vi "VirtualATE_V2.vi"() -> ()   [LabVIEW 2026]
uses:
  <vilib>/NI/Modbus Library/API/Modbus API.lvclass/Modbus API.ctl
  <vilib>/NI/Modbus Library/Transmission Data Unit/Transmission Data Unit.lvclass/Transmission Data Unit.ctl
  <vilib>/NI/Modbus Library/Transmission Data Unit/Write Unit ID.vi
  <vilib>/NI/Modbus Library/API/Read Transmission Data Unit.vi
  <vilib>/NI/Modbus Library/API/Write Transmission Data Unit.vi
  <vilib>/NI/Modbus Library/API/Master/Modbus Master.lvclass
  C:/Program Files/National Instruments/LabVIEW 2026/vi.lib/NI/Modbus Library/API/Modbus API.lvclass
  <vilib>/NI/Modbus Library/API/Wrapper/Create TCP Master.vi
  <vilib>/NI/Modbus Library/API/Wrapper/API Main.lvlib
panel:
  out "PLC_HB_TIMEOUT":bool
  out "PLC_HB_AGE_MS":u32
  out "PLC_LIVE_OK":bool
  out "STATE_ELAPSED_MS":u32
  out "처리 메시지":string
  out "ATE_READY":bool
  out "ACTIVE_RESULT":u16
  out "ACTIVE_ID":u16
  out "ATE_STATE":u16
  out "PLC_LIVE_COUNTER":u16
  out "PLC_ACCEPTED_ID":u16
  out "PLC_RX_RESPONSE_ID":u16
  out "PLC_RX_DONE":u16
  out "PLC_RX_RESULT":u16
  in  "검사 결과 선택":enum16{"PASS", "FAIL", "RETEST"}(ring)
  out "바깥 Tick Count(ms)":u32
  in  "ATE 읽기 정지":bool
  out "ALARM_CODE":u16
  out "SEQ_STATE":u16
  out "TEEST_RESULT_LATCH":u16
  out "ATE_DONE":u16
  out "ATE_RESPONSE_ID":u16
  out "ATE_RESULT":u16
  out "ATE_REQUEST_ID":u16
  out "ATE_REQUEST":u16
  out "마지막 Modbus 읽기 정상":bool
  out "수신 레지스터":u16[](array[numeric])
  out "error out":errorcluster
  in  "Unit ID":u8
  in  "Port":u16
  in  "Server IP":string
  # "0 ATE_LINK_TEST\n1 ATE_REQUEST\n2 ATE_REQUEST_ID\n3 ATE_RESULT\n4 ATE_RESPONSE_ID\n5 ATE_DONE\n6 TEST_RESULT_LATCH\n7 SEQ_STATE\n8 ALARM_CODE"
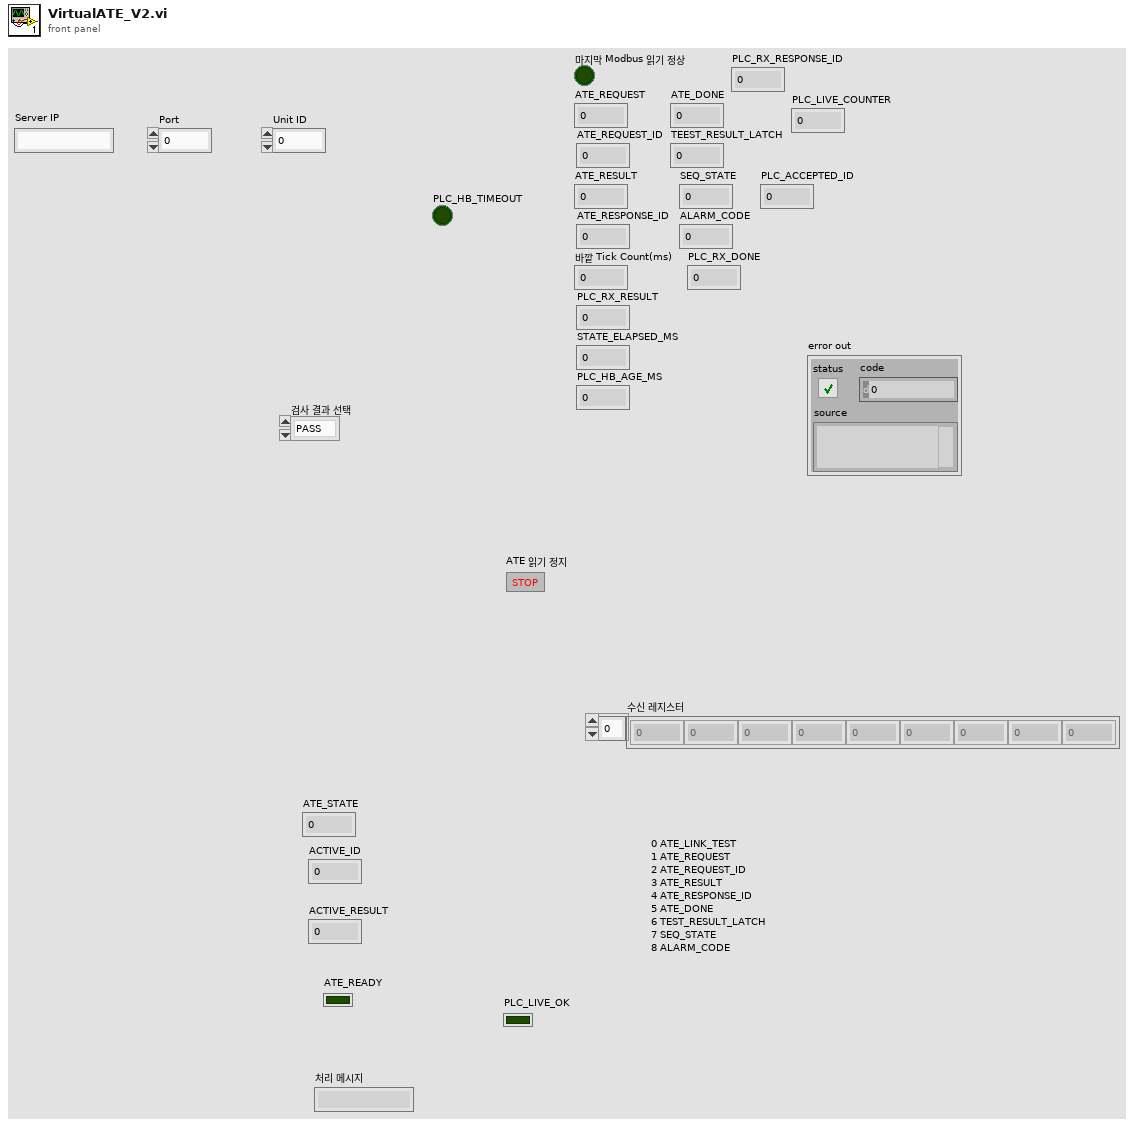
[diagram p1: front panel]
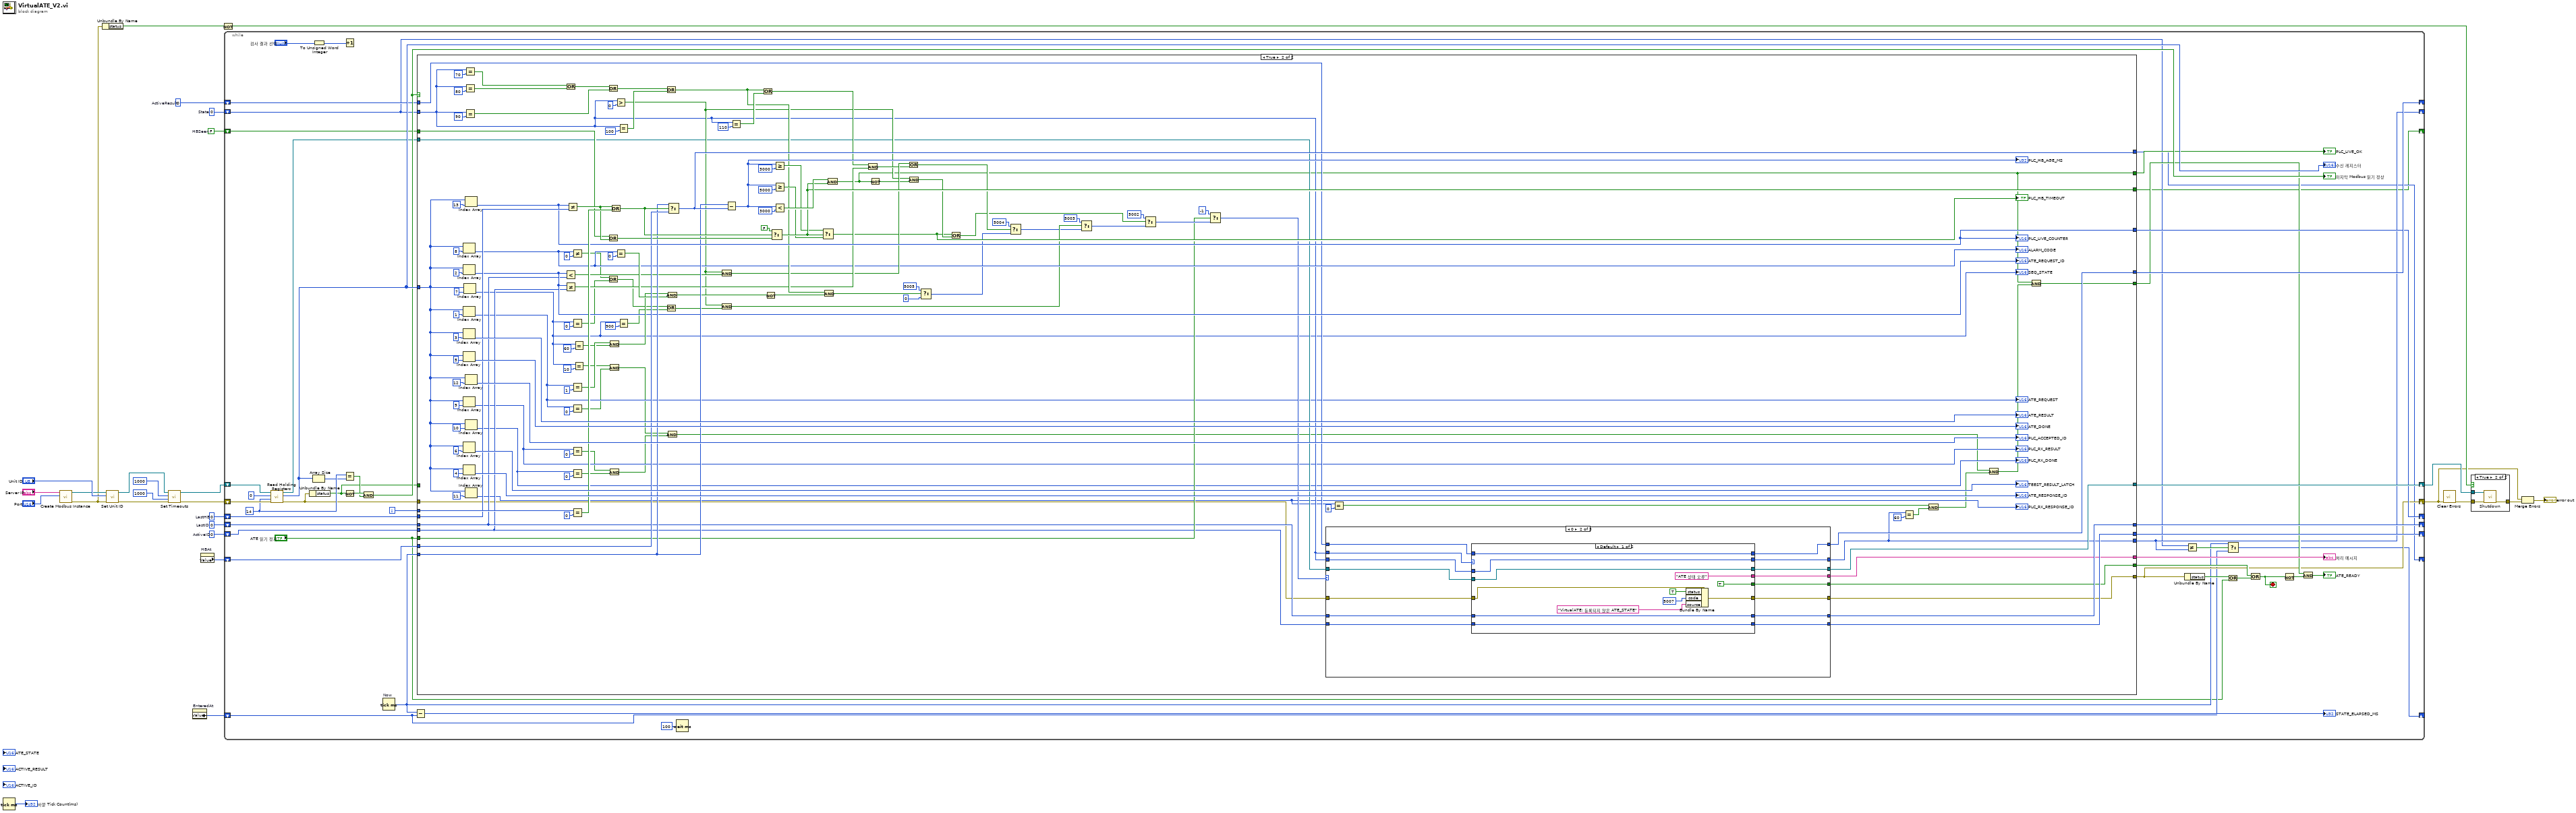
[diagram p0: block diagram]
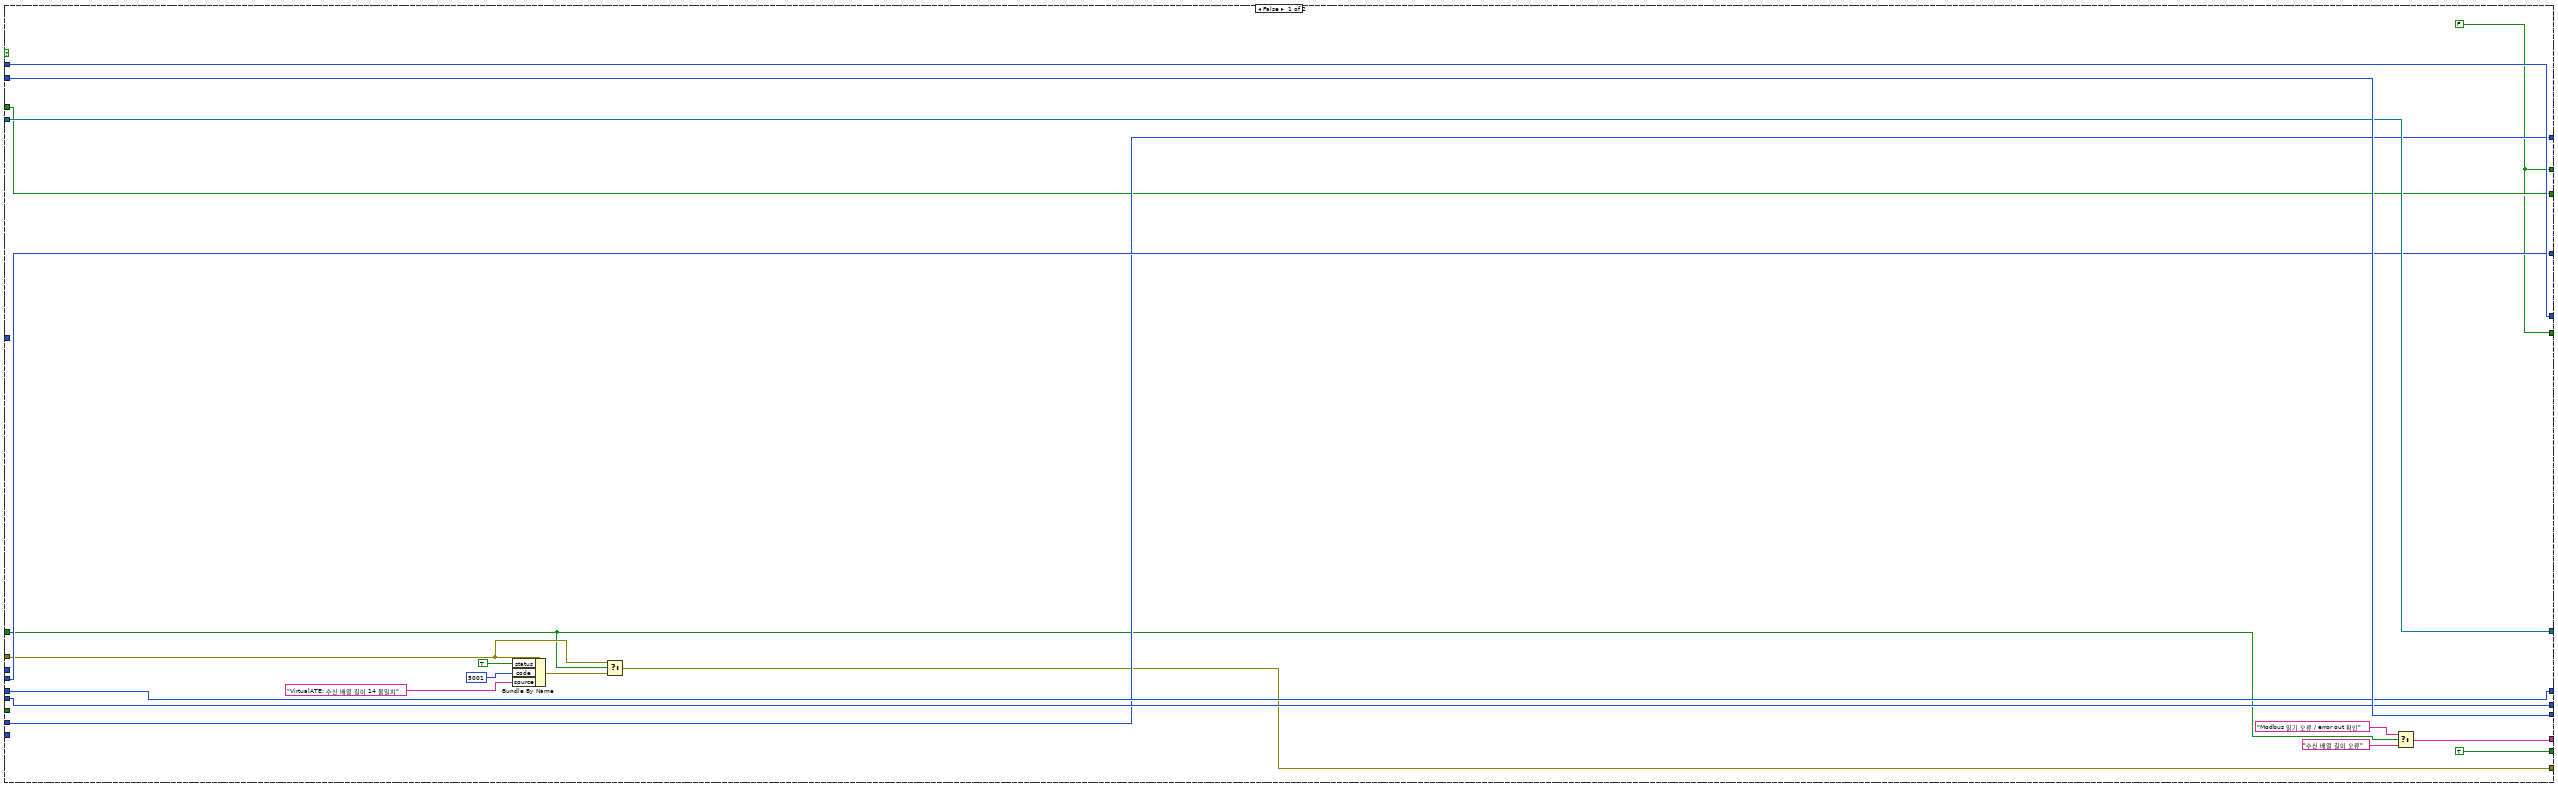
[diagram p3: hidden frame]
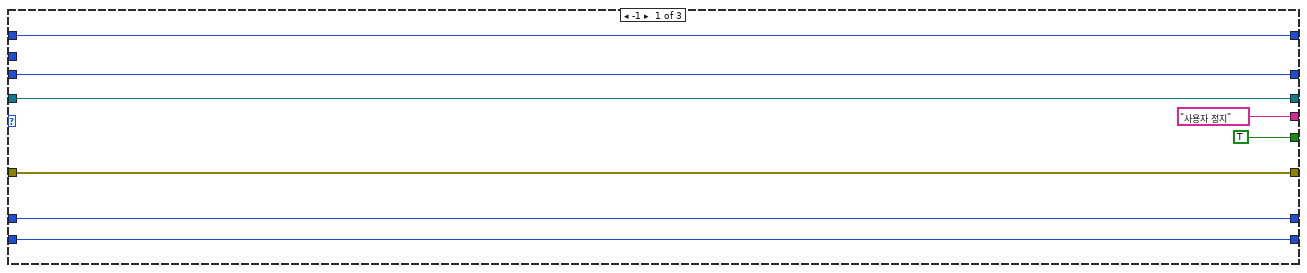
[diagram p4: hidden frame]
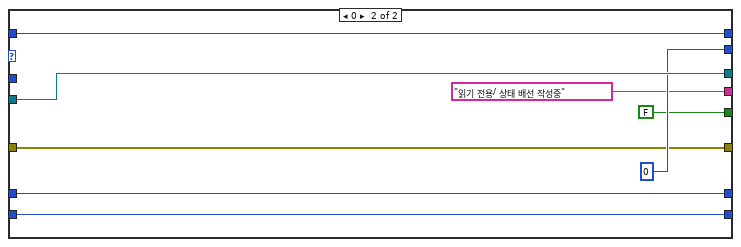
[diagram p5: hidden frame]
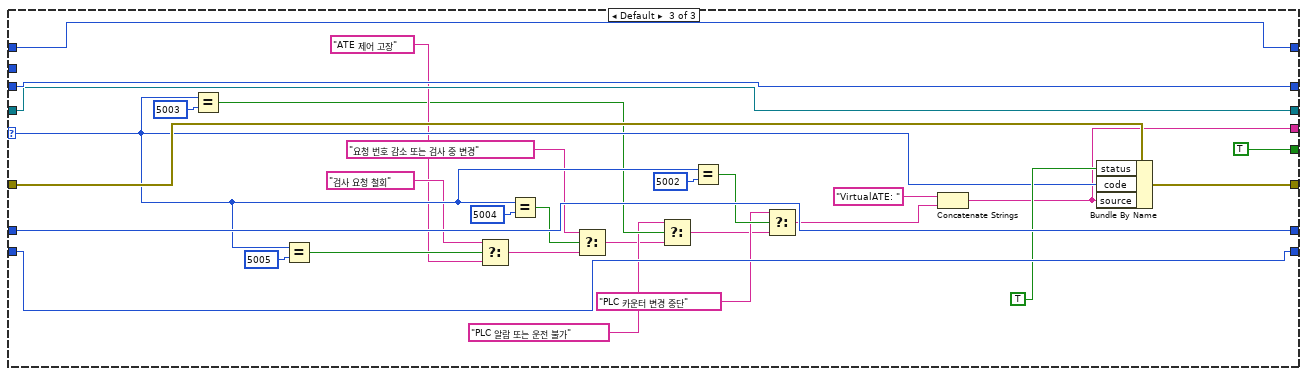
[diagram p6: hidden frame]
diagram:
  w9 = FALSE  # HBSeen
  w4 = u16 0  # LastHB
  w5 = u16 0  # ActiveResult
  w6 = u16 0  # ActiveID
  w7 = u16 0  # LastID
  w8 = u16 0  # State
  n1 = Tick Count (ms)() -> (millisecond timer value=→"바깥 Tick Count(ms)":u32)
  n2 = call-poly <vilib>:"Create Modbus Instance.vi"("port (502)"="Port", "address"="Server IP") -> ("error out"=w17:errorcluster, "TCP master instance"=w22:refnum<class "Modbus Master.lvclass">)  [unwired: 8 in]
  n3 = Unbundle By Name(w17) -> ("status"=w16:bool)
  n4 = call <vilib>:"Set Unit ID.vi"("error in"=w17, "unit ID"="Unit ID", "Modbus master in"=w22) -> ("error out"=w20:errorcluster, "Modbus master out"=w21:refnum<class "Modbus Master.lvclass">)  [unwired: 7 in]
  n5 = call <vilib>:"Set Timeouts.vi"("error in"=w20, "write operation timeout"=1000, "read operation timeout"=1000, "Modbus master in"=w21) -> ("error out"=w18:errorcluster, "Modbus master out"=w19:refnum<class "Modbus Master.lvclass">)  [unwired: 6 in]
  n6 = property on="EnteredAt" class="DigNum (strict)"() -> ("Value"=w2:u32)  [unwired: 2 in, 2 out]
  n7 = property on="HBAt" class="DigNum (strict)"() -> ("Value"=w1:u32)  [unwired: 2 in, 2 out]
  n8 = Not(x=w16) -> (.not. x?=w15:bool)
  n9 = while {
    shift-right: [w42] -> w11
    shift-left: w18 -> [w71]
    shift-right: [w54] -> w14
    shift-left: w19 -> [w72]
    shift-right: [w34] -> _
    shift-left: w8 -> [w33]
    shift-right: [w60] -> _
    shift-left: w7 -> [w61]
    shift-right: [w58] -> _
    shift-left: w6 -> [w59]
    shift-right: [w56] -> _
    shift-left: w5 -> [w57]
    shift-right: [w31] -> _
    shift-left: w1 -> [w50]
    shift-right: [w51] -> _
    shift-left: w4 -> [w52]
    shift-right: [w36] -> _
    shift-left: w2 -> [w32]
    shift-right: [w30] -> _
    shift-left: w9 -> [w49]
    i -> [w37]
    stop <- w39 stop-if-true
    w70 = u16 14 ("number of inputs")
    n10 = call-dynamic "Read Holding Registers.vi"("error in"=w71, "number of inputs"=w70, "starting address"=u16 0, "Modbus master in"=w72) -> ("error out"=w53:errorcluster, "register values"=w66:u16[], "Modbus master out"=w55:refnum<class "Modbus Master.lvclass">)  [unwired: 5 in]
    "수신 레지스터" <- w66
    n11 = Unbundle By Name(w53) -> ("status"=w48:bool)
    n12 = Array Size(array=w66) -> (size(s)=w69:i32)
    n13 = To Unsigned Word Integer(number="검사 결과 선택") -> (unsigned 16bit integer=w64:u16)
    n14 = Increment(x=w64) -> ()  [unwired: 1 out]
    n15 = Equal?(x=w70, y=w69) -> (x = y?=w67:bool)
    n16 = Not(x=w48) -> (.not. x?=w68:bool)
    n17 = And(x=w68, y=w67) -> (x .and. y?=w65:bool)
    "마지막 Modbus 읽기 정상" <- w65
    n18 = Tick Count (ms) "Now"() -> (millisecond timer value=w29:u32)
    n19 = Subtract(x=w29, y=w32) -> (x-y=→"STATE_ELAPSED_MS":u32)
    n20 = case shown="True" w65 {
      tunnel: w66 -> [_ w218]
      tunnel: w33 -> [w94 w120]
      tunnel: [w94 w109] -> w34
      tunnel: w61 -> [w93 w132]
      tunnel: [w93 w131] -> w60
      tunnel: w59 -> [w92 w130]
      tunnel: [w92 w129] -> w58
      tunnel: w57 -> [w91 w128]
      tunnel: [w91 w127] -> w56
      tunnel: w55 -> [w90 w126]
      tunnel: [w90 w125] -> w54
      tunnel: w53 -> [w82 w124]
      tunnel: [w76 w123] -> w42
      tunnel: w52 -> [w89 w209]
      tunnel: [w89 w205] -> w51
      tunnel: w50 -> [w88 w203]
      tunnel: [w88 w204] -> w31
      tunnel: w49 -> [w87 w206]
      tunnel: [w87 w193] -> w30
      tunnel: w48 -> [w80 _]
      tunnel: [TRUE w121] -> w46
      tunnel: [w77 w122] -> w45
      tunnel: [w75 w95] -> w43
      tunnel: [w75 w96] -> w38
      tunnel: w37 -> [_ w211]
      tunnel: w29 -> [_ w197]
      tunnel: "ATE 읽기 정지" -> [_ w134]
      frame False {
        w75 = FALSE
        n21 = Bundle By Name(cluster=w82, "status"=TRUE, "code"=5001, "source"="VirtualATE: 수신 배열 길이 14 불일치") -> (w83:errorcluster)
        n22 = Select(t=w82, s=w80, f=w83) -> (s? t:f=w76:errorcluster)
        n23 = Select(t="Modbus 읽기 오류 / error out 확인", s=w80, f="수신 배열 길이 오류") -> (s? t:f=w77:string)
      }
      frame True {
        n24 = Index Array(array=w218, index=3) -> (element=→"ATE_RESULT":u16)
        n25 = Index Array(array=w218, index=5) -> (element=→"ATE_DONE":u16)
        n26 = Index Array(array=w218, index=6) -> (element=→"TEEST_RESULT_LATCH":u16)
        n27 = Index Array(array=w218, index=4) -> (element=→"ATE_RESPONSE_ID":u16)
        n28 = Index Array(array=w218, index=8) -> (element=w161:u16)
        "ALARM_CODE" <- w161
        n29 = Index Array(array=w218, index=2) -> (element=w167:u16)
        "ATE_REQUEST_ID" <- w167
        n30 = Index Array(array=w218, index=1) -> (element=w117:u16)
        "ATE_REQUEST" <- w117
        n31 = Index Array(array=w218, index=9) -> (element=w115:u16)
        "PLC_RX_RESULT" <- w115
        n32 = Index Array(array=w218, index=7) -> (element=w119:u16)
        "SEQ_STATE" <- w119
        n33 = Equal?(x=w120, y=u16 70) -> (x = y?=w185:bool)
        n34 = Equal?(x=w120, y=u16 80) -> (x = y?=w184:bool)
        n35 = Equal?(x=w120, y=u16 90) -> (x = y?=w183:bool)
        n36 = Index Array(array=w218, index=13) -> (element=w205:u16)
        "PLC_LIVE_COUNTER" <- w205
        n37 = Index Array(array=w218, index=12) -> (element=→"PLC_ACCEPTED_ID":u16)
        n38 = Index Array(array=w218, index=10) -> (element=w113:u16)
        "PLC_RX_DONE" <- w113
        n39 = Index Array(array=w218, index=11) -> (element=w111:u16)
        "PLC_RX_RESPONSE_ID" <- w111
        n40 = Or(x=w185, y=w184) -> (x .or. y?=w182:bool)
        n41 = Less?(x=w167, y=w132) -> (x < y?=w166:bool)
        n42 = Not Equal?(x=w167, y=w130) -> (x != y?=w164:bool)
        n43 = Not Equal?(x=w205, y=w209) -> (x != y?=w207:bool)
        n44 = Not Equal?(x=w161, y=u16 0) -> (x != y?=w157:bool)
        n45 = Equal?(x=w119, y=u16 0) -> (x = y?=w156:bool)
        n46 = Equal?(x=w117, y=u16 1) -> (x = y?=w174:bool)
        n47 = Equal?(x=w117, y=u16 0) -> (x = y?=w106:bool)
        n48 = Equal?(x=w115, y=u16 0) -> (x = y?=w105:bool)
        n49 = Equal?(x=w113, y=u16 0) -> (x = y?=w104:bool)
        n50 = Equal?(x=w211, y=0) -> (x = y?=w208:bool)
        n51 = Equal?(x=w119, y=u16 60) -> (x = y?=w173:bool)
        n52 = Equal?(x=w119, y=u16 10) -> (x = y?=w107:bool)
        n53 = Or(x=w182, y=w183) -> (x .or. y?=w180:bool)
        n54 = Or(x=w206, y=w207) -> (x .or. y?=w202:bool)
        n55 = Or(x=w157, y=w156) -> (x .or. y?=w155:bool)
        n56 = And(x=w174, y=w173) -> (x .and. y?=w171:bool)
        n57 = And(x=w107, y=w106) -> (x .and. y?=w101:bool)
        n58 = And(x=w105, y=w104) -> (x .and. y?=w100:bool)
        n59 = Or(x=w207, y=w208) -> (x .or. y?=w201:bool)
        n60 = Greater?(x=w120, y=u16 0) -> (0:w152:bool)
        n61 = Equal?(x=w161, y=u16 0) -> (x = y?=w172:bool)
        n62 = Equal?(x=w120, y=u16 100) -> (x = y?=w181:bool)
        n63 = Equal?(x=w119, y=u16 900) -> (x = y?=w154:bool)
        n64 = Or(x=w180, y=w181) -> (x .or. y?=w168:bool)
        n65 = Or(x=w155, y=w154) -> (x .or. y?=w153:bool)
        n66 = And(x=w171, y=w172) -> (x .and. y?=w170:bool)
        n67 = And(x=w101, y=w100) -> (x .and. y?=w98:bool)
        n68 = Select(t=w197, s=w201, f=w203) -> (s? t:f=w204:u32)
        n69 = And(x=w152, y=w166) -> (x .and. y?=w163:bool)
        n70 = And(x=w152, y=w153) -> (x .and. y?=w144:bool)
        n71 = Subtract(x=w197, y=w204) -> (x-y=w196:u32)
        "PLC_HB_AGE_MS" <- w196
        n72 = Equal?(x=w120, y=u16 110) -> (x = y?=w178:bool)
        n73 = Or(x=w168, y=w178) -> (x .or. y?=w165:bool)
        n74 = Not(x=w170) -> (.not. x?=w169:bool)
        n75 = Select(t=FALSE, s=w201, f=w202) -> (s? t:f=w193:bool)
        n76 = Greater Or Equal?(x=w196, y=u32 3000) -> (x >= y?=w192:bool)
        n77 = Greater Or Equal?(x=w196, y=u32 5000) -> (x >= y?=w191:bool)
        n78 = Less?(x=w196, y=u32 3000) -> (x < y?=w199:bool)
        n79 = Select(t=w192, s=w193, f=w191) -> (s? t:f=w149:bool)
        "PLC_HB_TIMEOUT" <- w149
        n80 = And(x=w168, y=w169) -> (x .and. y?=w148:bool)
        n81 = And(x=w199, y=w193) -> (x .and. y?=w96:bool)
        n82 = And(x=w165, y=w164) -> (x .and. y?=w162:bool)
        n83 = Not(x=w96) -> (.not. x?=w151:bool)
        n84 = Or(x=w163, y=w162) -> (x .or. y?=w145:bool)
        n85 = And(x=w152, y=w151) -> (x .and. y?=w150:bool)
        n86 = Select(t=5005, s=w148, f=0) -> (s? t:f=w141:i32)
        n87 = Or(x=w149, y=w150) -> (x .or. y?=w143:bool)
        n88 = Select(t=5004, s=w145, f=w141) -> (s? t:f=w140:i32)
        n89 = Select(t=5003, s=w144, f=w140) -> (s? t:f=w138:i32)
        n90 = Select(t=5002, s=w143, f=w138) -> (s? t:f=w136:i32)
        n91 = Select(t=-1, s=w134, f=w136) -> (s? t:f=w133:i32)
        n92 = case shown="0" w133 {
          selector: w133 -> [_ _ w294]
          tunnel: w120 -> [w238 w240 w302]
          tunnel: [w238 w247 w302] -> w109
          tunnel: w132 -> [w237 w253 w301]
          tunnel: [w237 w244 w301] -> w131
          tunnel: w130 -> [w236 w252 w300]
          tunnel: [w236 w243 w300] -> w129
          tunnel: [w235 w249 w299] -> w127
          tunnel: w128 -> [w235 w251 w299]
          tunnel: [w234 w248 w298] -> w125
          tunnel: w126 -> [w234 w250 w298]
          tunnel: [w233 w246 w297] -> w123
          tunnel: w124 -> [w233 w245 w296]
          tunnel: ["사용자 정지" w241 w275] -> w122
          tunnel: [TRUE w242 TRUE] -> w121
          tunnel: w120 -> [_ w239 _]
          frame -1 {
          }
          frame 0 {
            n93 = case shown="Default" w239 {
              tunnel: w253 -> [w254 w269]
              tunnel: w252 -> [w255 w268]
              tunnel: w251 -> [w264 w273]
              tunnel: w250 -> [w263 w272]
              tunnel: [w264 w273] -> w249
              tunnel: [w263 w272] -> w248
              tunnel: [w265 u16 0] -> w247
              tunnel: [w258 w270] -> w246
              tunnel: w245 -> [w262 w270]
              tunnel: [w254 w269] -> w244
              tunnel: [w255 w268] -> w243
              tunnel: [TRUE FALSE] -> w242
              tunnel: ["ATE 상태 오류" "읽기 전용/ 상태 배선 작성중"] -> w241
              tunnel: w240 -> [w265 _]
              frame Default {
                n94 = Bundle By Name(cluster=w262, "status"=TRUE, "code"=5007, "source"="VirtualATE: 등록되지 않은 ATE_STATE") -> (w258:errorcluster)
              }
              frame 0 {
              }
            }
          }
          frame Default {
            n95 = Equal?(x=w294, y=5003) -> (x = y?=w285:bool)
            n96 = Equal?(x=w294, y=5005) -> (x = y?=w289:bool)
            n97 = Select(t="검사 요청 철회", s=w289, f="ATE 제어 고장" ("t")) -> (s? t:f=w280:string)
            n98 = Equal?(x=w294, y=5004) -> (x = y?=w286:bool)
            n99 = Select(t="요청 번호 감소 또는 검사 중 변경", s=w286, f=w280) -> (s? t:f=w279:string)
            n100 = Select(t="PLC 알람 또는 운전 불가", s=w285, f=w279) -> (s? t:f=w278:string)
            n101 = Equal?(x=w294, y=5002) -> (x = y?=w284:bool)
            n102 = Select(t="PLC 카운터 변경 중단", s=w284, f=w278) -> (s? t:f=w276:string)
            n103 = Concatenate Strings("VirtualATE: ", w276) -> (w275:string)
            n104 = Bundle By Name(cluster=w296, "status"=TRUE, "code"=w294, "source"=w275) -> (w297:errorcluster)
          }
        }
        n105 = Equal?(x=w111, y=u16 0) -> (x = y?=w103:bool)
        n106 = Equal?(x=w109, y=u16 60) -> (x = y?=w102:bool)
        n107 = And(x=w103, y=w102) -> (x .and. y?=w99:bool)
        n108 = And(x=w98, y=w99) -> (x .and. y?=w97:bool)
        n109 = And(x=w96, y=w97) -> (x .and. y?=w95:bool)
      }
    }
    "처리 메시지" <- w45
    "PLC_LIVE_OK" <- w38
    n110 = Wait (ms)(milliseconds to wait=u32 100) -> ()  [unwired: 1 out]
    n111 = Unbundle By Name(w42) -> ("status"=w41:bool)
    n112 = Not Equal?(x=w33, y=w34) -> (x != y?=w35:bool)
    n113 = Or(x=w41, y="ATE 읽기 정지") -> (x .or. y?=w47:bool)
    n114 = Select(t=w29, s=w35, f=w32) -> (s? t:f=w36:u32)
    n115 = Or(x=w46, y=w47) -> (x .or. y?=w39:bool)
    n116 = Not(x=w39) -> (.not. x?=w40:bool)
    n117 = And(x=w43, y=w40) -> (x .and. y?=→"ATE_READY":bool)
  }
  n118 = call <vilib>:"Clear Errors.vi"("error in (no error)"=w11) -> ("error out"=w10:errorcluster)  [unwired: 5 in, 1 out]
  n119 = case shown="True" w15 {
    tunnel: w14 -> [_ w306]
    tunnel: [w303 w305] -> w13
    tunnel: w10 -> [w303 w304]
    frame False {
    }
    frame True {
      n120 = call-dynamic "Shutdown.vi"("error in"=w304, "Modbus master in"=w306) -> ("error out"=w305:errorcluster)  [unwired: 9 in]
    }
  }
  n121 = Merge Errors(w11, w13) -> (→"error out":errorcluster)
